vi "Set_Operation_Mode.vi"(8 "error in (no error)":errorcluster, 10 "Motor Control Mode":T1, 11 "WEG_SCA06_Modbus in":refnum<class "WEG_SCA06_Modbus.lvclass">) -> (0 "error out":errorcluster, 3 "WEG_SCA06_Modbus out":refnum<class "WEG_SCA06_Modbus.lvclass">)   [LabVIEW 2021, in "WEG_SCA06_Modbus.lvclass"]
doc: "This VI set the motor control mode between Speed (RPM) and Torque (N.m)"
uses:
  WEG_SCA06_Modbus.lvclass
  Motor/Type_Defs/Control_Mode.ctl
  WEG_SCA06_Modbus.lvclass/WEG_SCA06_Modbus.ctl
  Modbus_Master/Modbus_Master.lvclass
  Motor/Motor.lvclass
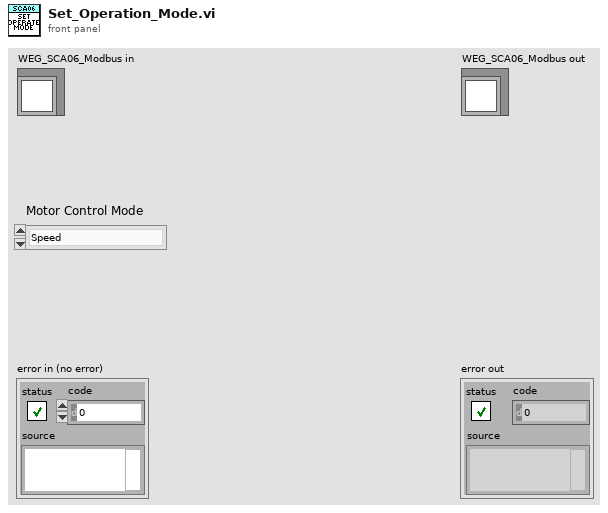
[diagram p1: front panel]
types:
  T1 = typedef "Motor.lvclass/Control_Mode.ctl" = enum16{"Speed", "Torque"}
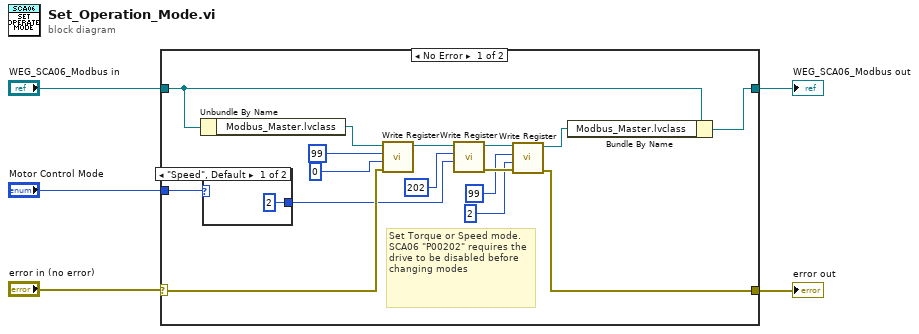
[diagram p0: block diagram]
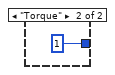
[diagram p2: hidden frame]
diagram:
  n1 = case shown="No Error" "error in (no error)" {
    selector: "error in (no error)" -> [w18 w24]
    tunnel: "WEG_SCA06_Modbus in" -> [w20 w25]
    tunnel: [w19 w25] -> w3
    tunnel: [w10 w24] -> w2
    tunnel: "Motor Control Mode" -> [w7 _]
    frame No Error {
      # "Set Torque or Speed mode.\nSCA06 \"P00202\" requires the drive to be disabled before changing modes"
      n2 = Unbundle By Name(w20) -> ("Modbus_Master.lvclass"=w21:refnum<class "Modbus_Master.lvclass">)
      n3 = case shown="\"Speed\", Default" w7 {
        tunnel: [u16 2 ("Value") u16 1 ("Value")] -> w6
        frame "Speed", Default {
        }
        frame "Torque" {
        }
      }
      n4 = call "Write Register.vi"("error in (no error)"=w18, "Value"=u16 0, "Register Address"=u16 99, "Modbus_Master in"=w21) -> ("Modbus_Master out"=w15:refnum<class "Modbus_Master.lvclass">)  [unwired: 6 in, 1 out]
      n5 = call "Write Register.vi"("Value"=w6, "Register Address"=u16 202, "Modbus_Master in"=w15) -> ("error out"=w12:errorcluster, "Modbus_Master out"=w13:refnum<class "Modbus_Master.lvclass">)  [unwired: 7 in]
      n6 = call "Write Register.vi"("error in (no error)"=w12, "Value"=u16 2, "Register Address"=u16 99, "Modbus_Master in"=w13) -> ("error out"=w10:errorcluster, "Modbus_Master out"=w11:refnum<class "Modbus_Master.lvclass">)  [unwired: 6 in]
      n7 = Bundle By Name(cluster=w20, "Modbus_Master.lvclass"=w11) -> (w19:refnum<class "WEG_SCA06_Modbus.lvclass">)
    }
    frame Error {
    }
  }
  "error out" <- w2
  "WEG_SCA06_Modbus out" <- w3
